vi "Run.vi"(8 "error in (no error)":errorcluster, 11 "TCS in":refnum<class "TCS.lvclass">) -> (0 "error out":errorcluster, 3 "TCS out":refnum<class "TCS.lvclass">)   [LabVIEW 2018, in "TCS.lvclass"]
uses:
  TCS.lvclass
  TCS.lvclass/TCS.ctl
  State Machine/State Machine.lvclass/State Machine.ctl
  State Machine/State Machine.lvclass
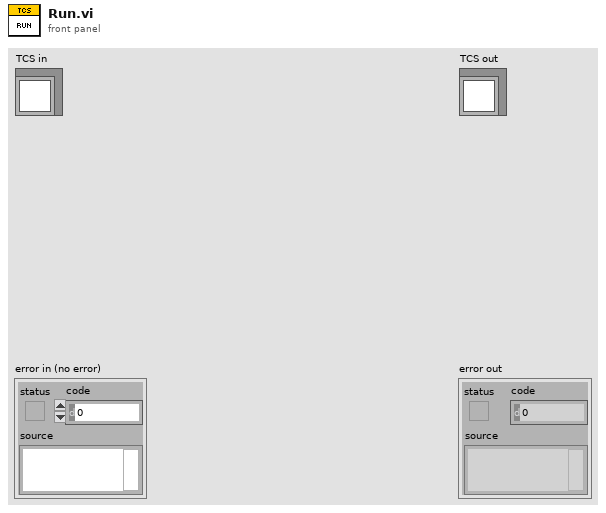
[diagram p1: front panel]
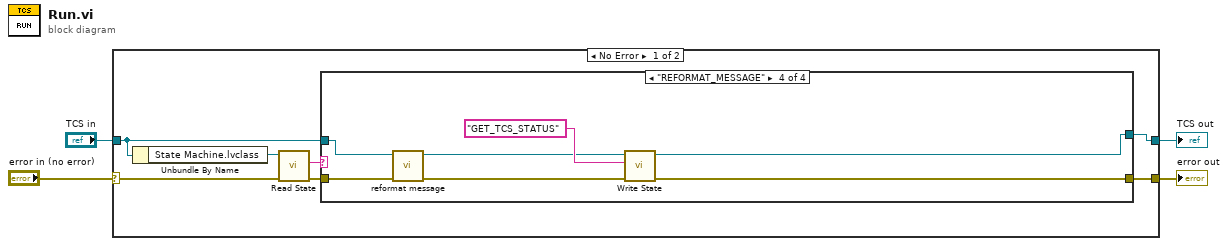
[diagram p0: block diagram]
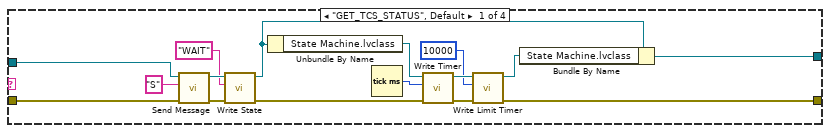
[diagram p2: hidden frame]
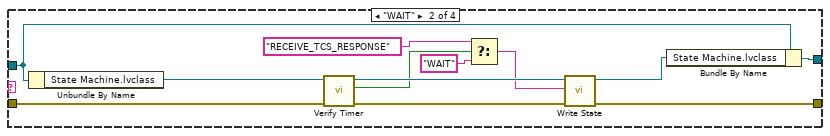
[diagram p3: hidden frame]
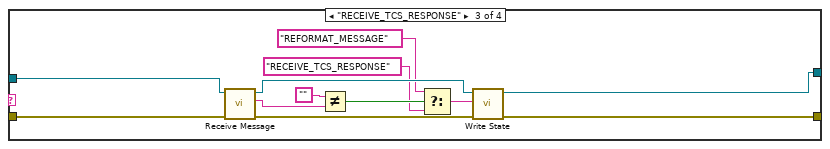
[diagram p4: hidden frame]
diagram:
  n1 = case shown="No Error" "error in (no error)" {
    selector: "error in (no error)" -> [w10 w60]
    tunnel: [w5 w60] -> w3
    tunnel: [w6 w59] -> w1
    tunnel: "TCS in" -> [w8 w59]
    frame No Error {
      n2 = Unbundle By Name(w8) -> ("State Machine.lvclass"=w11:refnum<class "State Machine.lvclass">)
      n3 = call-dynamic "Read State.vi"("error in (no error)"=w10, "State Machine in"=w11) -> ("error out"=w7:errorcluster, "State"=w9:string)  [unwired: 7 in, 1 out]
      n4 = case shown="\"REFORMAT_MESSAGE\"" w9 {
        tunnel: w8 -> [w27 w39 w51 w58]
        tunnel: w7 -> [w26 w36 w49 w56]
        tunnel: [w20 w38 w50 w57] -> w6
        tunnel: [w17 w34 w48 w55] -> w5
        frame "GET_TCS_STATUS", Default {
          n5 = call "Send Message.vi"("error in (no error)"=w26, "message"="S", "TCS in"=w27) -> ("error out"=w23:errorcluster, "TCS out"=w24:refnum<class "TCS.lvclass">)  [unwired: 7 in]
          n6 = call "Write State.vi"("error in (no error)"=w23, "State"="WAIT" ("message"), "TCS in"=w24) -> ("error out"=w14:errorcluster, "TCS out"=w21:refnum<class "TCS.lvclass">)  [unwired: 7 in]
          n7 = Unbundle By Name(w21) -> ("State Machine.lvclass"=w15:refnum<class "State Machine.lvclass">)
          n8 = Tick Count (ms)() -> (millisecond timer value=w12:u32)
          n9 = call "Write Timer.vi"("error in (no error)"=w14, "Timer"=w12, "State Machine in"=w15) -> ("error out"=w16:errorcluster, "State Machine out"=w19:refnum<class "State Machine.lvclass">)  [unwired: 7 in]
          n10 = call "Write Limit Timer.vi"("error in (no error)"=w16, "Limit Timer"=10000, "State Machine in"=w19) -> ("error out"=w17:errorcluster, "State Machine out"=w18:refnum<class "State Machine.lvclass">)  [unwired: 7 in]
          n11 = Bundle By Name(cluster=w21, "State Machine.lvclass"=w18) -> (w20:refnum<class "TCS.lvclass">)
        }
        frame "WAIT" {
          n12 = Unbundle By Name(w39) -> ("State Machine.lvclass"=w37:refnum<class "State Machine.lvclass">)
          n13 = call "Verify Timer.vi"("error in (no error)"=w36, "State Machine in"=w37) -> ("error out"=w32:errorcluster, "time out"=w30:bool, "State Machine out"=w33:refnum<class "State Machine.lvclass">)  [unwired: 7 in]
          n14 = Select(t="RECEIVE_TCS_RESPONSE", s=w30, f="WAIT") -> (s? t:f=w31:string)
          n15 = call-dynamic "Write State.vi"("error in (no error)"=w32, "State"=w31, "State Machine in"=w33) -> ("error out"=w34:errorcluster, "State Machine out"=w35:refnum<class "State Machine.lvclass">)  [unwired: 7 in]
          n16 = Bundle By Name(cluster=w39, "State Machine.lvclass"=w35) -> (w38:refnum<class "TCS.lvclass">)
        }
        frame "RECEIVE_TCS_RESPONSE" {
          n17 = call "Receive Message.vi"("error in (no error)"=w49, "TCS in"=w51) -> ("error out"=w47:errorcluster, "Message"=w44:string, "TCS out"=w46:refnum<class "TCS.lvclass">)  [unwired: 7 in]
          n18 = Not Equal?(x="", y=w44) -> (x != y?=w45:bool)
          n19 = Select(t="REFORMAT_MESSAGE", s=w45, f="RECEIVE_TCS_RESPONSE") -> (s? t:f=w40:string)
          n20 = call "Write State.vi"("error in (no error)"=w47, "State"=w40, "TCS in"=w46) -> ("error out"=w48:errorcluster, "TCS out"=w50:refnum<class "TCS.lvclass">)  [unwired: 7 in]
        }
        frame "REFORMAT_MESSAGE" {
          n21 = call "reformat message.vi"("error in (no error)"=w56, "TCS in"=w58) -> ("error out"=w53:errorcluster, "TCS out"=w52:refnum<class "TCS.lvclass">)  [unwired: 8 in]
          n22 = call "Write State.vi"("error in (no error)"=w53, "State"="GET_TCS_STATUS", "TCS in"=w52) -> ("error out"=w55:errorcluster, "TCS out"=w57:refnum<class "TCS.lvclass">)  [unwired: 7 in]
        }
      }
    }
    frame Error {
    }
  }
  "error out" <- w3
  "TCS out" <- w1
